vi "RemoteVI Demo.vi"() -> ()   [LabVIEW 2020]
doc: "Demo of the RemoteVI toolkit. Publishes its own front panel with RemoteVI Start.vi (VI unwired, so the caller - this VI - is published on port 8088 - NI Application Web Server often holds 8080), runs a 50 ms loop that draws a moving sine (amplitude Numeric) on the graph until Stop is pressed, then calls RemoteVI Stop.vi. Ask opens a LabVIEW Two Button Dialog and shows the answer in Answer; Open File opens the native file dialog and shows the chosen file's name in File - both are answered from the browser like the panel is operated (docs\\protocol.md section 7). Open URL in a browser to see and operate the panel."
uses:
  source/RemoteVI.lvlib
panel:
  out "error out":errorcluster
  out "File":string
  out "Answer":string
  out "URL":string
  in  "Open File":bool
  in  "Ask":bool
  out "Sine":dbl[](graph)
  in  "Message":string="Hello from LabVIEW"
  in  "Enable":bool
  in  "Mode":i32(ring) items=["Off", "Slow", "Fast"]
  in  "Numeric":dbl=6.0
  in  "Stop":bool
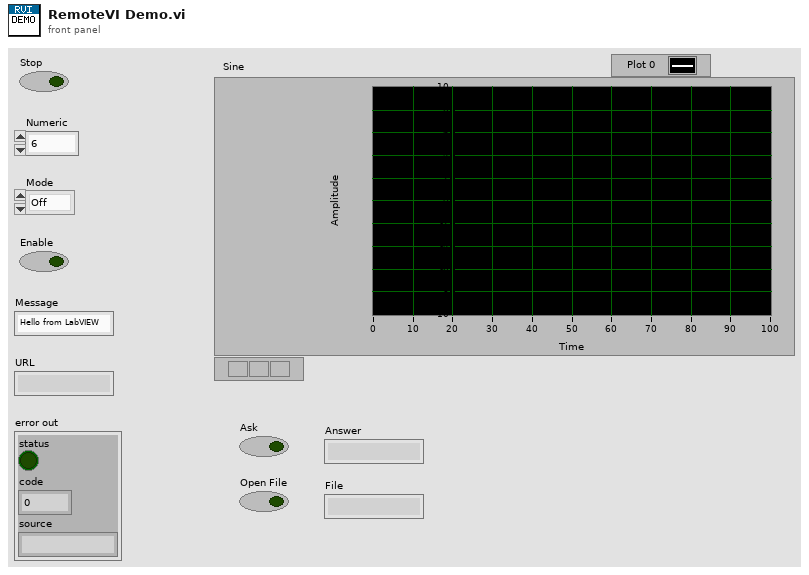
[diagram p1: front panel]
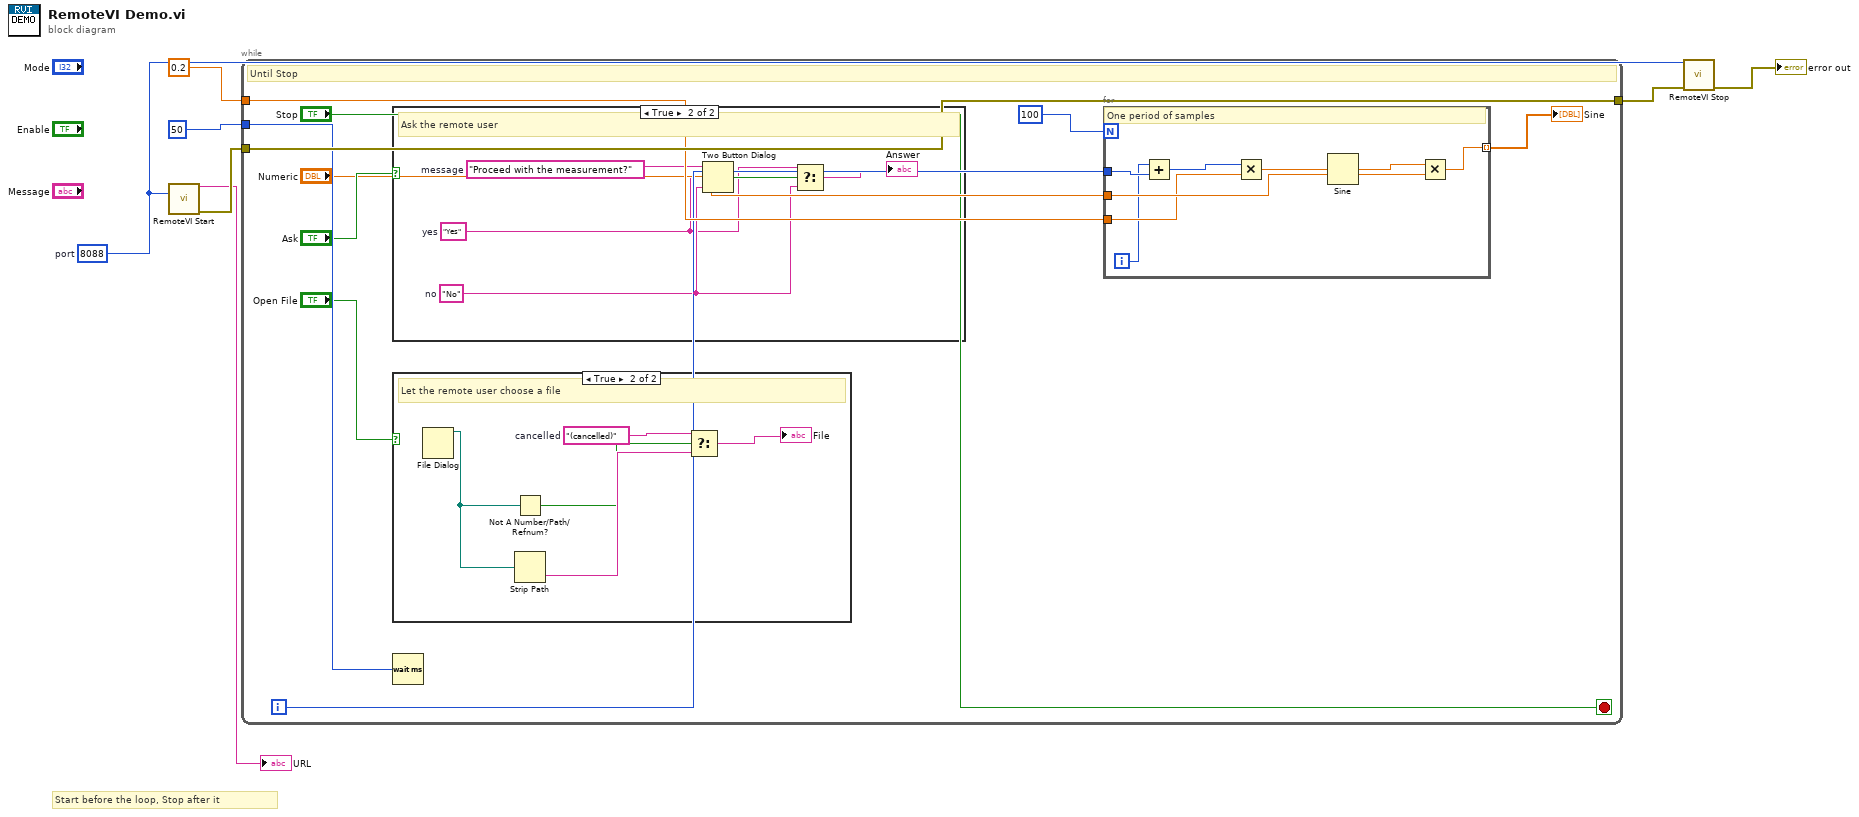
[diagram p0: block diagram]
diagram:
  w2 = u16 8088  # port
  # "Start before the loop, Stop after it"
  n1 = call "RemoteVI Start.vi"("port"=w2) -> ("URL"=→"URL":string, "error out"=w3:errorcluster)  [unwired: 13 in]
  n2 = while {
    tunnel: 0.2 -> [w14]
    tunnel: 50 -> [w15]
    tunnel: w3 -> [w16]
    tunnel: [w16] -> w6
    i -> [w13]
    stop <- "Stop" stop-if-true
    # "Until Stop"
    n3 = case shown="True" "Ask" {
      frame False {
        # "Nothing to ask"
      }
      frame True {
        w25 = "No"  # no
        w24 = "Yes"  # yes
        w23 = "Proceed with the measurement?"  # message
        # "Ask the remote user"
        n4 = Two Button Dialog(message=w23, 1:w25, 2:w24) -> (T button?=w26:bool)
        n5 = Select(t=w24, s=w26, f=w25) -> (s? t:f=→"Answer":string)
      }
    }
    n6 = case shown="True" "Open File" {
      frame False {
        # "Nothing to open"
      }
      frame True {
        w21 = "(cancelled)"  # cancelled
        # "Let the remote user choose a file"
        n7 = File Dialog() -> (3:w18:path)  [unwired: 7 in, 3 out]
        n8 = Not A Number/Path/Refnum?(number/path/refnum=w18) -> (NaN/Path/Refnum?=w19:bool)
        n9 = Strip Path(path=w18) -> (name=w20:string)  [unwired: 1 out]
        n10 = Select(t=w21, s=w19, f=w20) -> (s? t:f=→"File":string)
      }
    }
    n11 = Wait (ms)(milliseconds to wait=w15) -> ()  [unwired: 1 out]
    n12 = for {
      N: 100 -> [_]
      tunnel: w13 -> [w29]
      tunnel: "Numeric" -> [w31]
      tunnel: w14 -> [w30]
      tunnel: [w35] -> w10 mode=indexing
      i -> [w28]
      # "One period of samples"
      n13 = Add(x=w28, y=w29) -> (x+y=w32:i32)
      n14 = Multiply(x=w32, y=w30) -> (x*y=w33:dbl)
      n15 = Sine(x=w33) -> (sin(x)=w34:dbl)
      n16 = Multiply(x=w34, y=w31) -> (x*y=w35:dbl)
    }
    "Sine" <- w10
  }
  n17 = call "RemoteVI Stop.vi"("port"=w2, "error in"=w6) -> ("error out"=→"error out":errorcluster)  [unwired: 13 in]
